vi "P2_ExecutionState.vi"(11 "Inputs":string[](array[string])) -> (2 "Output/Failure":string, 3 "CLI Process Return Code":i32)   [LabVIEW 2026]
doc: "Slice 1.1 probe: Open VI Reference, read Execution State, Close Reference."
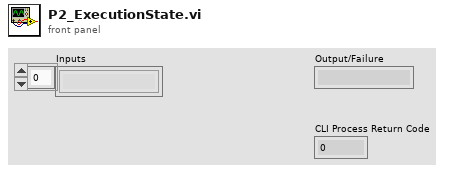
[diagram p1: front panel]
types:
  T1 = enum32{"Bad", "Idle", "Run top level", "Running"}
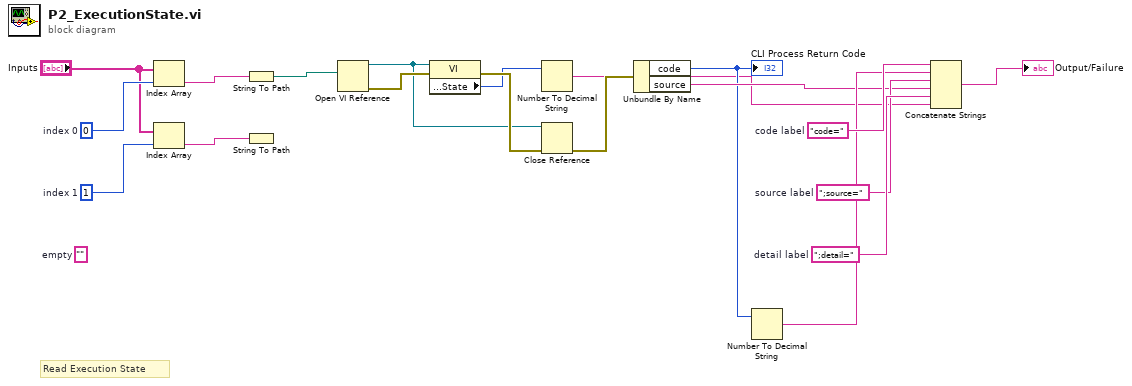
[diagram p0: block diagram]
diagram:
  w18 = ";detail="  # detail label
  w17 = ";source="  # source label
  w16 = "code="  # code label
  (unwired) ""  # empty
  w3 = 1  # index 1
  w2 = 0  # index 0
  # "Read Execution State"
  n1 = Index Array(array="Inputs", index=w2) -> (element=w4:string)
  n2 = Index Array(array="Inputs", index=w3) -> (element=w5:string)
  n3 = String To Path(string=w4) -> (path=w6:path)
  n4 = String To Path(string=w5) -> ()  [unwired: 1 out]
  n5 = Open VI Reference(vi path=w6) -> (vi reference=w7:refnum<vi>, error out=w8:errorcluster)  [unwired: 5 in]
  n6 = property class="VI"(reference=w7, error in=w8) -> (error out=w10:errorcluster, "Execution:State"=w9:T1)  [unwired: 1 out]
  n7 = Number To Decimal String(number=w9) -> (decimal integer string=w11:string)  [unwired: 1 in]
  n8 = Close Reference(reference=w7, error in (no error)=w10) -> (error out=w12:errorcluster)
  n9 = Unbundle By Name(w12) -> ("code"=w13:i32, "source"=w14:string)
  "CLI Process Return Code" <- w13
  n10 = Number To Decimal String(number=w13) -> (decimal integer string=w15:string)  [unwired: 1 in]
  n11 = Concatenate Strings(w16, w15, w17, w14, w18, w11) -> (→"Output/Failure":string)
